vi "Event Hits.vi"(8 "other":i32, 9 "stock":i32, 10 "candidate":i32, 11 "scope":T1(ring)) -> (2 "as other?":bool, 3 "as stock?":bool)   [LabVIEW 2020, in "Full Featured MCP Server.lvlib"]
doc: "Tells whether an event hits one particular stock. As the stock of the event: when it is that stock (scope one stock or two stocks), a stock of the same sector (scope sector), or always (scope market). As the other stock: only with the scope two stocks, when it is the second stock of the event."
uses:
  Full Featured MCP Server.lvlib
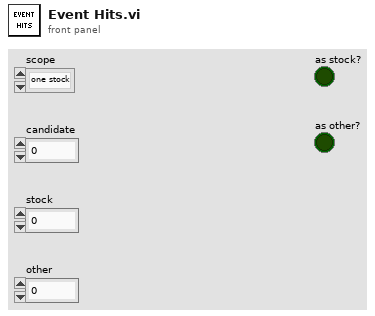
[diagram p1: front panel]
types:
  T1 = enum16{"one stock", "two stocks", "sector", "market"}
  T2 = cluster{"name":string, "sector":i32, "quality":i32, "start price":dbl, "drift":dbl, "volatility":dbl, "beta":dbl, "jumpiness":dbl, "description":string}[]
  T3 = cluster{"name":string, "sector":i32, "quality":i32, "start price":dbl, "drift":dbl, "volatility":dbl, "beta":dbl, "jumpiness":dbl, "description":string}
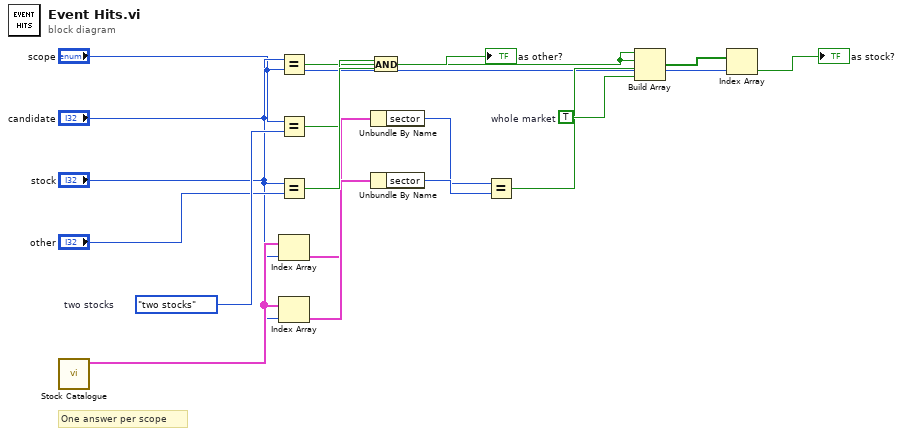
[diagram p0: block diagram]
diagram:
  w15 = T1."two stocks"  # two stocks
  w12 = TRUE  # whole market
  # "One answer per scope"
  n1 = call "Stock Catalogue.vi"() -> ("stocks"=w5:T2)  [unwired: 10 in, 1 out]
  n2 = Equal?(x="candidate", y="stock") -> (x = y?=w6:bool)
  n3 = Equal?(x="scope", y=w15) -> (x = y?=w16:bool)
  n4 = Equal?(x="candidate", y="other") -> (x = y?=w17:bool)
  n5 = Index Array(array=w5, index="candidate") -> (element=w7:T3)
  n6 = Index Array(array=w5, index="stock") -> (element=w9:T3)
  n7 = And(x=w16, y=w17) -> (x .and. y?=→"as other?":bool)
  n8 = Unbundle By Name(w7) -> ("sector"=w8:i32)
  n9 = Unbundle By Name(w9) -> ("sector"=w10:i32)
  n10 = Equal?(x=w8, y=w10) -> (x = y?=w11:bool)
  n11 = Build Array(w6, w6, w11, w12) -> (w13:bool[])
  n12 = Index Array(array=w13, index="scope") -> (element=→"as stock?":bool)
